vi "get target by index.vi"(8 "error in":errorcluster, 10 "index":i32, 11 "system hierarchy":T1) -> (0 "error out":errorcluster, 3 "target hierarchy":T1)   [LabVIEW 2013, in "PL_Serialization Interface.lvlib"]
doc: "Searches a flattened instance data hierarhy for a specific target by the index, assuming that the current root element is the system level. This function makes no assurances that the target returned will be the one you were looking for, and it is better to locate the target by its unique identifier. If the target is not found, error 538508 is returned."
uses:
  PL_Serialization Interface.lvlib
  <vilib>/NI/Configuration Framework/tree serializer/flat hierarchy.ctl
  <vilib>/NI/Configuration Framework/tree serializer/full hierarchy.ctl
  <vilib>/NI/Configuration Framework/tree serializer/hierarchy element.ctl
  <vilib>/NI/Configuration Framework/tree serializer/instance data.ctl
  <vilib>/NI/Configuration Framework/tree serializer/NISE_CEF_TreeSerializer.lvlib
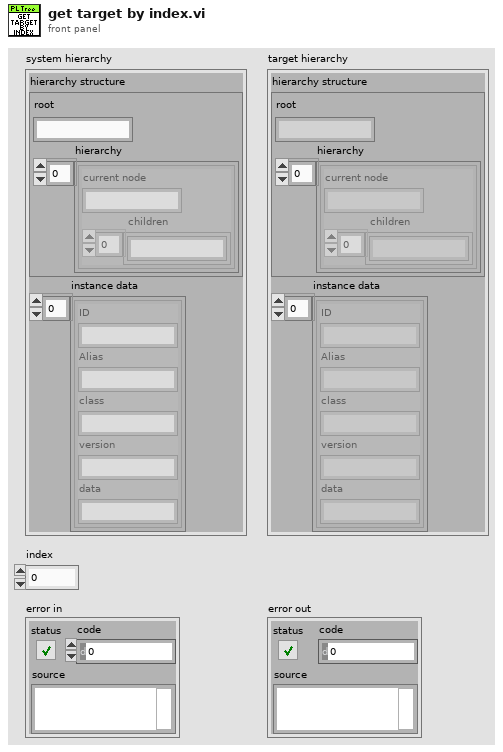
[diagram p1: front panel]
types:
  T1 = typedef "NISE_CEF_TreeSerializer.lvlib/flat hierarchy.ctl" = cluster{"hierarchy structure":T2, "instance data":T4[]}
  T2 = typedef "NISE_CEF_TreeSerializer.lvlib/full hierarchy.ctl" = cluster{"root":string, "hierarchy":T3[]}
  T3 = typedef "NISE_CEF_TreeSerializer.lvlib/hierarchy element.ctl" = cluster{"current node":string, "children":string[]}
  T4 = typedef "NISE_CEF_TreeSerializer.lvlib/instance data.ctl" = cluster{"ID":string, "Alias":string, "class":string, "version":string, "data":string}
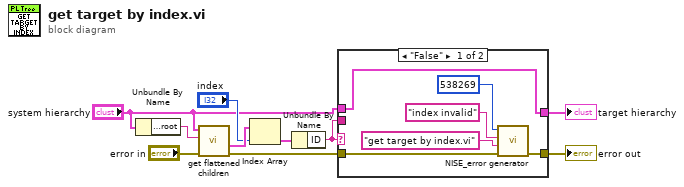
[diagram p0: block diagram]
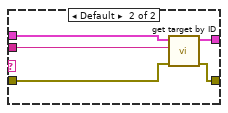
[diagram p2: hidden frame]
diagram:
  n1 = Unbundle By Name("system hierarchy") -> ("hierarchy structure.root"=w2:string)
  n2 = call <vilib>:"get flattened children.vi"("error in"="error in", "ID"=w2, "flat hierarchy"="system hierarchy") -> ("error out"=w4:errorcluster, "children"=w7:T4[])  [unwired: 7 in]
  n3 = Index Array(array=w7, index="index") -> (element=w5:T4)
  n4 = Unbundle By Name(w5) -> ("ID"=w1:string)
  n5 = case shown="\"False\"" w1 {
    tunnel: [w14 w21] -> w10
    tunnel: w1 -> [_ w20]
    tunnel: [w16 w19] -> w9
    tunnel: w4 -> [w15 w18]
    tunnel: "system hierarchy" -> [w16 w17]
    frame "False" {
      n6 = call <vilib>:"NISE_error generator.vi"("error in"=w15, "source"="get target by index.vi", "append error message"="index invalid", "error code (0)"=538269) -> ("error out"=w14:errorcluster)  [unwired: 5 in]
    }
    frame Default {
      n7 = call "get target by ID.vi"("error in"=w18, "UID"=w20, "full system"=w17) -> ("error out"=w21:errorcluster, "target hierarchy"=w19:T1)  [unwired: 7 in]
    }
  }
  "error out" <- w10
  "target hierarchy" <- w9
